vi "RemoteVI System Color.vi"(0 "nIndex":i32=13) -> (4 "rgb":u32)   [LabVIEW 2020, in "RemoteVI.lvlib"]
doc: "A Windows display colour (user32 GetSysColor nIndex - 13 COLOR_HIGHLIGHT, 4 COLOR_MENU) as a LabVIEW pixmap value 0x00RRGGBB, the order RemoteVI Capture Window.vi returns pixels in (GetSysColor answers a COLORREF 0x00BBGGRR). Win32 only."
uses:
  RemoteVI.lvlib
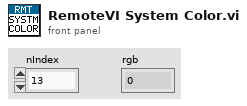
[diagram p1: front panel]
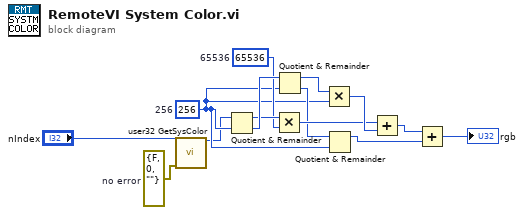
[diagram p0: block diagram]
diagram:
  w5 = u32 65536  # 65536
  w4 = u32 256  # 256
  w2 = errorcluster {"status"=FALSE, "code"=0, "source"=""}  # no error
  n1 = call "user32 GetSysColor.vi"("nIndex"="nIndex", "error in"=w2) -> ("color"=w3:u32)  [unwired: 12 in, 1 out]
  n2 = Quotient & Remainder(x=w3, y=w4) -> (x-y*floor(x/y)=w6:u32, floor(x/y)=w7:u32)
  n3 = Multiply(x=w6, y=w5) -> (x*y=w11:u32)
  n4 = Quotient & Remainder(x=w7, y=w4) -> (x-y*floor(x/y)=w8:u32, floor(x/y)=w9:u32)
  n5 = Multiply(x=w8, y=w4) -> (x*y=w12:u32)
  n6 = Quotient & Remainder(x=w9, y=w4) -> (x-y*floor(x/y)=w10:u32)  [unwired: 1 out]
  n7 = Add(x=w11, y=w12) -> (x+y=w13:u32)
  n8 = Add(x=w13, y=w10) -> (x+y=→"rgb":u32)
